vi "VIH Project - Correct Master Rule.vi"(11 "Master Rule":T1) -> (3 "Master Rule out":T1)   [LabVIEW 2014]
doc: "::: VI Helpeks :::\nCopyright (c) 2000-2026 Konstantin Shifershteyn. All rights reserved."
uses:
  _VIH HelpGen.llb/VIH HelpGen Typedef - Cluster - Group Rule.ctl
  _VIH HelpGen.llb/VIH HelpGen Typedef - Enum - Default,Enable,Disable.ctl
  _VIH HelpGen.llb/VIH HelpGen Typedef - Cluster - Group Rule - Source Paths.ctl
  _VIH HelpGen.llb/VIH HelpGen Typedef - Cluster - Group Rule - Target Paths.ctl
  _VIH HelpGen.llb/VIH HelpGen Typedef - Enum - Description Mode.ctl
  _VIH HelpGen.llb/VIH HelpGen Typedef - Cluster - Control Rule.ctl
  _VIH HelpGen.llb/VIH HelpGen Typedef - Cluster - Enum Value Info.ctl
  _VIH HelpGen.llb/VIH HelpGen Typedef - Cluster - Group Rule - Flags.ctl
panel:
  # "VI Helpeks\nCopyright (c) 2012-2026 Konstantin Shifershteyn"
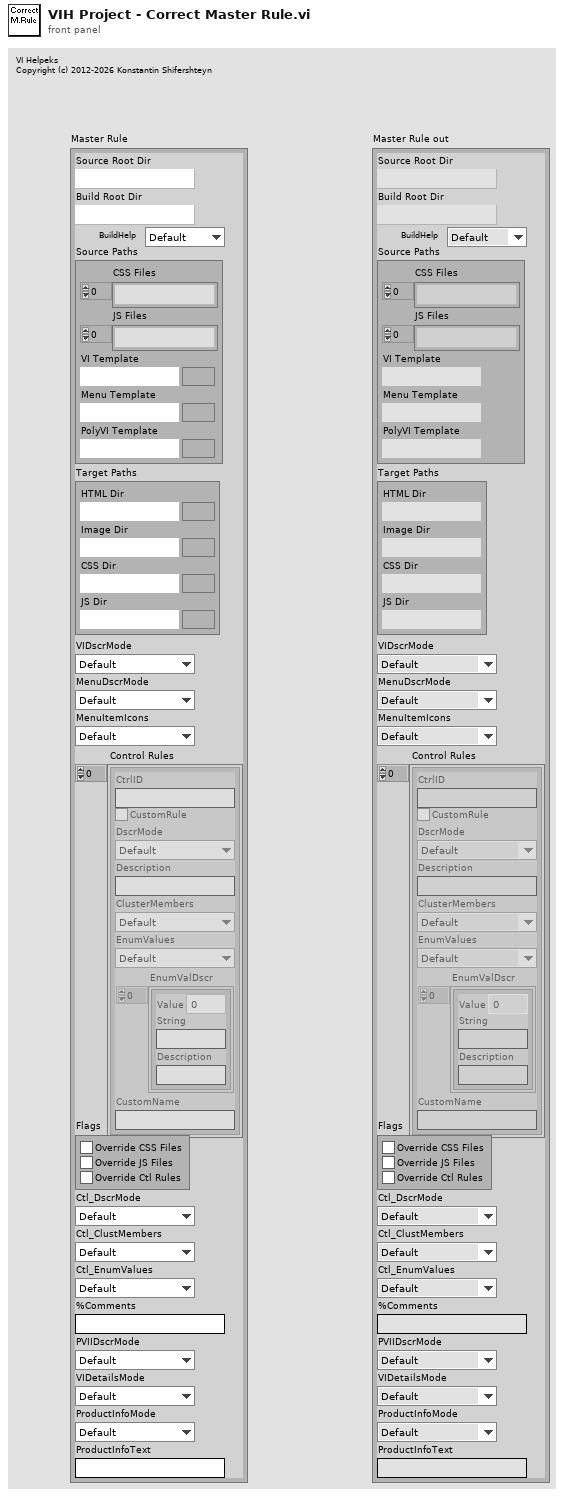
[diagram p1: front panel]
types:
  T1 = typedef "VIH HelpGen Typedef - Cluster - Group Rule.ctl" = cluster{"Source Root Dir":path, "Build Root Dir":path, "BuildHelp":T2, "Source Paths":T3, "Target Paths":T4, "VIDscrMode":T5, "MenuDscrMode":T5, "MenuItemIcons":T2, "Control Rules":T6[], "Flags":T8, "Ctl_DscrMode":T5, "Ctl_ClustMembers":T2, "Ctl_EnumValues":T2, "%Comments":string, "PVIIDscrMode":T5, "VIDetailsMode":T5, "ProductInfoMode":T2, "ProductInfoText":string}
  T2 = typedef "VIH HelpGen Typedef - Enum - Default,Enable,Disable.ctl" = enum16{"Default", "Enable", "Disable"}
  T3 = typedef "VIH HelpGen Typedef - Cluster - Group Rule - Source Paths.ctl" = cluster{"CSS Files":path[], "JS Files":path[], "VI Template":path, "Menu Template":path, "PolyVI Template":path}
  T4 = typedef "VIH HelpGen Typedef - Cluster - Group Rule - Target Paths.ctl" = cluster{"HTML Dir":path, "Image Dir":path, "CSS Dir":path, "JS Dir":path}
  T5 = typedef "VIH HelpGen Typedef - Enum - Description Mode.ctl" = enum16{"Default", "Description", "Description1", "Description2", "Custom", "None"}
  T6 = typedef "VIH HelpGen Typedef - Cluster - Control Rule.ctl" = cluster{"CtrlID":string, "CustomRule":bool, "DscrMode":T5, "Description":string, "ClusterMembers":T2, "EnumValues":T2, "EnumValDscr":T7[], "CustomName":string}
  T7 = typedef "VIH HelpGen Typedef - Cluster - Enum Value Info.ctl" = cluster{"Value":ext, "String":string, "Description":string}
  T8 = typedef "VIH HelpGen Typedef - Cluster - Group Rule - Flags.ctl" = cluster{"Override CSS Files":bool, "Override JS Files":bool, "Override Ctl Rules":bool}
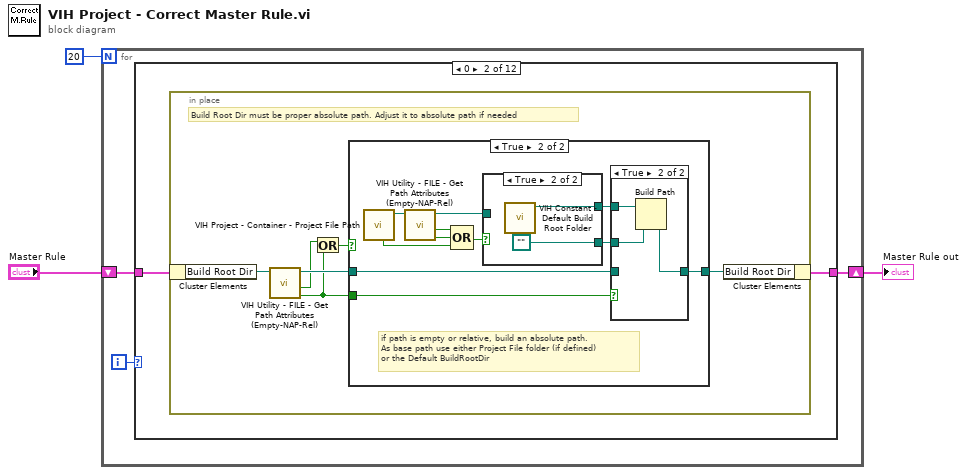
[diagram p0: block diagram]
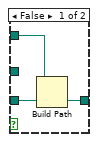
[diagram p4: hidden frame]
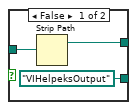
[diagram p5: hidden frame]
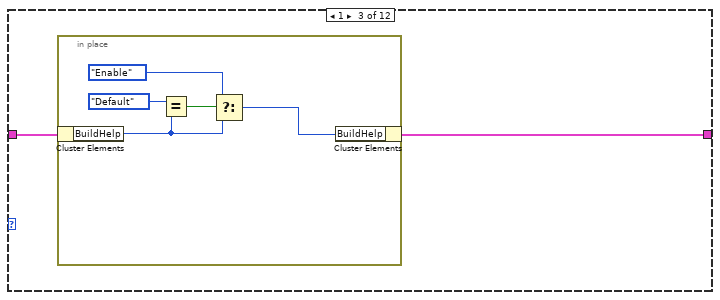
[diagram p6: hidden frame]
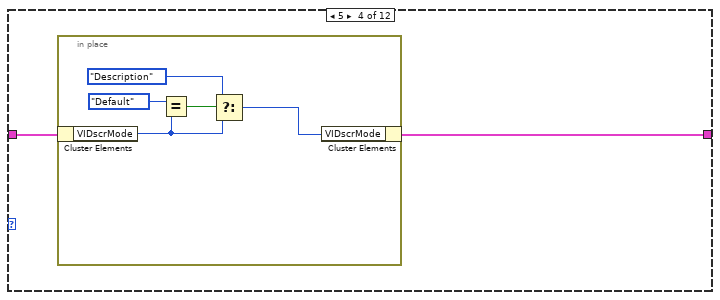
[diagram p7: hidden frame]
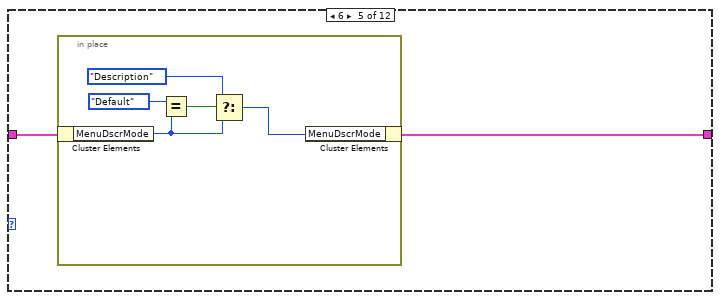
[diagram p8: hidden frame]
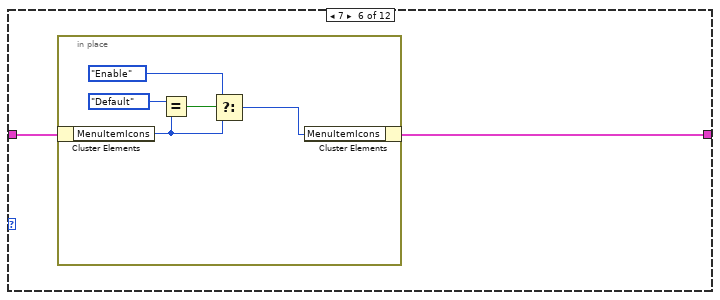
[diagram p9: hidden frame]
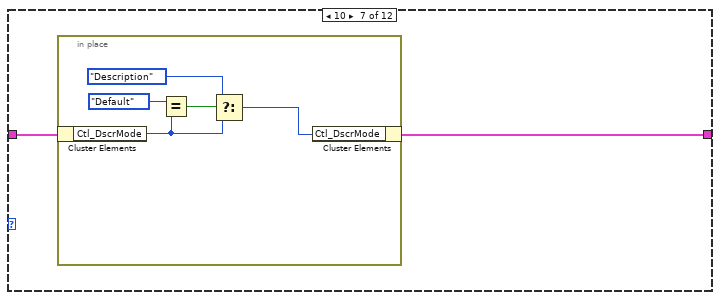
[diagram p10: hidden frame]
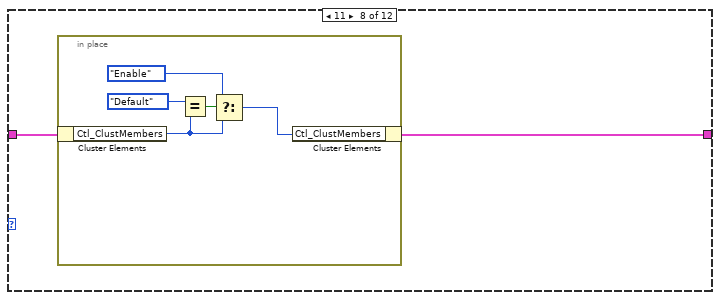
[diagram p11: hidden frame]
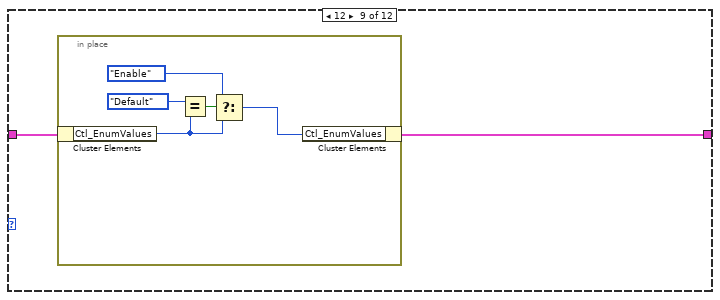
[diagram p12: hidden frame]
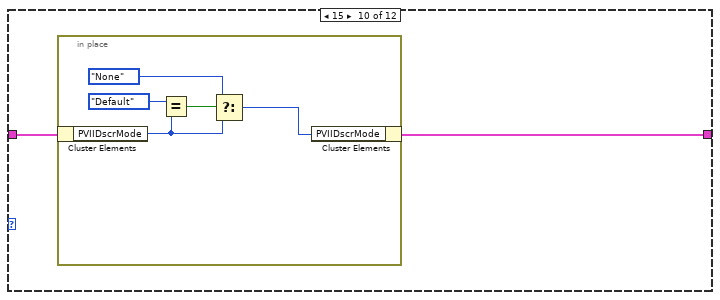
[diagram p13: hidden frame]
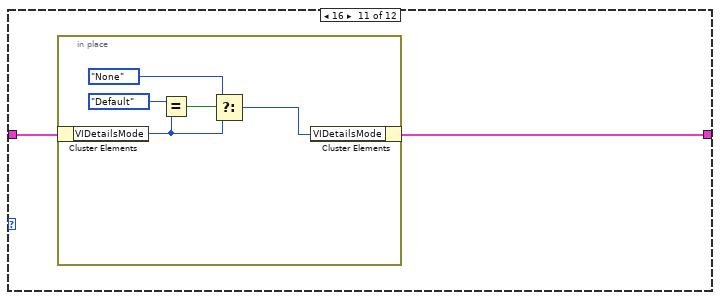
[diagram p14: hidden frame]
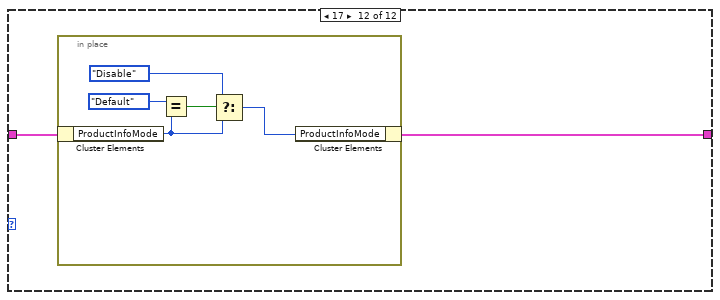
[diagram p15: hidden frame]
diagram:
  n1 = for {
    N: 20 -> [_]
    shift-right: [w4] -> w2
    shift-left: "Master Rule" -> [w5]
    i -> [w6]
    n2 = case shown="0" w6 {
      tunnel: w5 -> [w7 w9 w40 w47 w54 w61 w68 w75 w82 w89 w96 w103]
      tunnel: [w7 w8 w39 w46 w53 w60 w67 w74 w81 w88 w95 w102] -> w4
      frame Default {
      }
      frame 0 {
        n3 = in-place {
          # "Build Root Dir must be proper absolute path. Adjust it to absolute path if needed"
          n4 = in-place-cluster #1(w9) -> ("Build Root Dir"=w15:path)
          n5 = call "VIH Utility - FILE - Get Path Attributes (Empty-NAP-Rel).vi"("Path"=w15) -> ("Not A Path or Empty path"=w10:bool, "Relative path"=w12:bool, "dup Path"=w13:path)  [unwired: 6 in, 2 out]
          n6 = Or(x=w12, y=w10) -> (x .or. y?=w11:bool)
          n7 = case shown="True" w11 {
            tunnel: [w16 w26] -> w14
            tunnel: w13 -> [w16 w27]
            tunnel: w10 -> [_ w19]
            frame False {
              # "good absolute path"
            }
            frame True {
              # "if path is empty or relative, build an absolute path.\nAs base path use either Project File folder (if defined)\nor the Default BuildRootDir"
              n8 = call "VIH Project - Container - Project File Path.vi"() -> ("Project File Path"=w23:path, "It's example"=w18:bool)  [unwired: 9 in, 1 out]
              n9 = call "VIH Utility - FILE - Get Path Attributes (Empty-NAP-Rel).vi"("Path"=w23) -> ("Not A Path or Empty path"=w21:bool, "Relative path"=w22:bool, "dup Path"=w25:path)  [unwired: 6 in, 2 out]
              n10 = Compound Arithmetic op=OR(w22, w21, w18) -> (w24:bool)
              n11 = case shown="True" w24 {
                tunnel: w25 -> [w36 _]
                tunnel: [w35 w38] -> w20
                tunnel: [path "VIHelpeksOutput" path ""] -> w17
                frame False {
                  n12 = Strip Path(path=w36) -> (stripped path=w35:path)  [unwired: 1 out]
                }
                frame True {
                  n13 = call "VIH Constant - Default Build Root Folder.vi"() -> ("Default Build Root Folder"=w38:path)  [unwired: 11 in]
                }
              }
              n14 = case shown="True" w19 {
                tunnel: w27 -> [w30 _]
                tunnel: [w29 w32] -> w26
                tunnel: w20 -> [w28 w33]
                tunnel: w17 -> [_ w31]
                frame False {
                  n15 = Build Path(base path=w28, name or relative path=w30) -> (appended path=w29:path)
                }
                frame True {
                  n16 = Build Path(base path=w33, name or relative path=w31) -> (appended path=w32:path)
                }
              }
            }
          }
          n17 = in-place-cluster #1("Build Root Dir"=w14) -> (w8:T1)
        }
      }
      frame 1 {
        n18 = in-place {
          n19 = in-place-cluster #2(w40) -> ("BuildHelp"=w44:T2)
          n20 = Equal?(x=VIH_HelpGen_Typedef_-_Enum_-_Default,Enable,Disable."Default", y=w44) -> (x = y?=w45:bool)
          n21 = Select(t=VIH_HelpGen_Typedef_-_Enum_-_Default,Enable,Disable."Enable", s=w45, f=w44) -> (s? t:f=w43:T2)
          n22 = in-place-cluster #2("BuildHelp"=w43) -> (w39:T1)
        }
      }
      frame 5 {
        n23 = in-place {
          n24 = in-place-cluster #3(w47) -> ("VIDscrMode"=w51:T5)
          n25 = Equal?(x=VIH_HelpGen_Typedef_-_Enum_-_Description_Mode."Default", y=w51) -> (x = y?=w52:bool)
          n26 = Select(t=VIH_HelpGen_Typedef_-_Enum_-_Description_Mode."Description", s=w52, f=w51) -> (s? t:f=w50:T5)
          n27 = in-place-cluster #3("VIDscrMode"=w50) -> (w46:T1)
        }
      }
      frame 6 {
        n28 = in-place {
          n29 = in-place-cluster #4(w54) -> ("MenuDscrMode"=w58:T5)
          n30 = Equal?(x=VIH_HelpGen_Typedef_-_Enum_-_Description_Mode."Default", y=w58) -> (x = y?=w59:bool)
          n31 = Select(t=VIH_HelpGen_Typedef_-_Enum_-_Description_Mode."Description", s=w59, f=w58) -> (s? t:f=w57:T5)
          n32 = in-place-cluster #4("MenuDscrMode"=w57) -> (w53:T1)
        }
      }
      frame 7 {
        n33 = in-place {
          n34 = in-place-cluster #5(w61) -> ("MenuItemIcons"=w65:T2)
          n35 = Equal?(x=VIH_HelpGen_Typedef_-_Enum_-_Default,Enable,Disable."Default", y=w65) -> (x = y?=w66:bool)
          n36 = Select(t=VIH_HelpGen_Typedef_-_Enum_-_Default,Enable,Disable."Enable", s=w66, f=w65) -> (s? t:f=w64:T2)
          n37 = in-place-cluster #5("MenuItemIcons"=w64) -> (w60:T1)
        }
      }
      frame 10 {
        n38 = in-place {
          n39 = in-place-cluster #6(w68) -> ("Ctl_DscrMode"=w72:T5)
          n40 = Equal?(x=VIH_HelpGen_Typedef_-_Enum_-_Description_Mode."Default", y=w72) -> (x = y?=w73:bool)
          n41 = Select(t=VIH_HelpGen_Typedef_-_Enum_-_Description_Mode."Description", s=w73, f=w72) -> (s? t:f=w71:T5)
          n42 = in-place-cluster #6("Ctl_DscrMode"=w71) -> (w67:T1)
        }
      }
      frame 11 {
        n43 = in-place {
          n44 = in-place-cluster #7(w75) -> ("Ctl_ClustMembers"=w79:T2)
          n45 = Equal?(x=VIH_HelpGen_Typedef_-_Enum_-_Default,Enable,Disable."Default", y=w79) -> (x = y?=w80:bool)
          n46 = Select(t=VIH_HelpGen_Typedef_-_Enum_-_Default,Enable,Disable."Enable", s=w80, f=w79) -> (s? t:f=w78:T2)
          n47 = in-place-cluster #7("Ctl_ClustMembers"=w78) -> (w74:T1)
        }
      }
      frame 12 {
        n48 = in-place {
          n49 = in-place-cluster #8(w82) -> ("Ctl_EnumValues"=w86:T2)
          n50 = Equal?(x=VIH_HelpGen_Typedef_-_Enum_-_Default,Enable,Disable."Default", y=w86) -> (x = y?=w87:bool)
          n51 = Select(t=VIH_HelpGen_Typedef_-_Enum_-_Default,Enable,Disable."Enable", s=w87, f=w86) -> (s? t:f=w85:T2)
          n52 = in-place-cluster #8("Ctl_EnumValues"=w85) -> (w81:T1)
        }
      }
      frame 15 {
        n53 = in-place {
          n54 = in-place-cluster #9(w89) -> ("PVIIDscrMode"=w93:T5)
          n55 = Equal?(x=VIH_HelpGen_Typedef_-_Enum_-_Description_Mode."Default", y=w93) -> (x = y?=w94:bool)
          n56 = Select(t=VIH_HelpGen_Typedef_-_Enum_-_Description_Mode."None", s=w94, f=w93) -> (s? t:f=w92:T5)
          n57 = in-place-cluster #9("PVIIDscrMode"=w92) -> (w88:T1)
        }
      }
      frame 16 {
        n58 = in-place {
          n59 = in-place-cluster #10(w96) -> ("VIDetailsMode"=w100:T5)
          n60 = Equal?(x=VIH_HelpGen_Typedef_-_Enum_-_Description_Mode."Default", y=w100) -> (x = y?=w101:bool)
          n61 = Select(t=VIH_HelpGen_Typedef_-_Enum_-_Description_Mode."None", s=w101, f=w100) -> (s? t:f=w99:T5)
          n62 = in-place-cluster #10("VIDetailsMode"=w99) -> (w95:T1)
        }
      }
      frame 17 {
        n63 = in-place {
          n64 = in-place-cluster #11(w103) -> ("ProductInfoMode"=w107:T2)
          n65 = Equal?(x=VIH_HelpGen_Typedef_-_Enum_-_Default,Enable,Disable."Default", y=w107) -> (x = y?=w108:bool)
          n66 = Select(t=VIH_HelpGen_Typedef_-_Enum_-_Default,Enable,Disable."Disable", s=w108, f=w107) -> (s? t:f=w106:T2)
          n67 = in-place-cluster #11("ProductInfoMode"=w106) -> (w102:T1)
        }
      }
    }
  }
  "Master Rule out" <- w2
